vi "Temperature Limits.vi"() -> ()   [LabVIEW 2021]
panel:
  out "Lower Temp":dbl=45.0
  out "Upper Temp":dbl=50.0
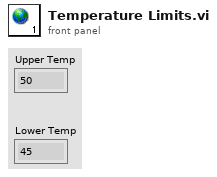
[diagram p1: front panel]
diagram:
